vi "DecodeSerializerEvents.vi"   [LabVIEW 2026]
uses:
  replay/Replay/src/Libraries/Replay/Replay.lvlib
  Launcher/Launcher.lvlib
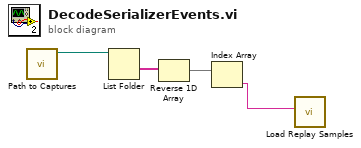
[diagram p0: block diagram]
diagram:
  n1 = call "Path to Captures.vi"() -> ("Captures"=w4:path)  [unwired: 11 in]
  n2 = List Folder(path=w4) -> (folder names=w3:string[])  [unwired: 3 in, 3 out]
  n3 = Reverse 1D Array(array=w3) -> (reversed array=w2:string[])
  n4 = Index Array(array=w2) -> (element=w1:string)  [unwired: 1 in]
  n5 = call "Load Replay Samples.vi"("Run ID"=w1) -> ()  [unwired: 9 in, 2 out]
